vi "Sequence-Start tracking.vi"   [LabVIEW 2020]
uses:
  Global Variables/gl_UI Ctrl Refs.vi
types:
  T1 = enum8{"Enabled", "Disabled", "Disabled and Grayed Out"}
  T2 = typedef "UI ctrl refs cluster.ctl" = cluster{"Top level VI path":path, "Top level VI ref":refnum<vi>, "User menu ref":refnum<k9>, "Sub Panel control":refnum<vi>, "Imaging Param Tab":refnum<vi>, "Occurrence-Start drivers":refnum<k4>, "Occurrence-Speed logging initialised":refnum<k4>, "Occurrence-XYZ stage initialised":refnum<k4>, "Exit button":refnum<vi>, "Status ind":refnum<vi>, "Set as origin":refnum<vi>, "Speed Logging":refnum<vi>, "Time Lapse":refnum<vi>, "Live Imaging":refnum<vi>, "AOL Z Stack":refnum<vi>, "Motor Z Stack":refnum<vi>, "Funct Acq button":refnum<vi>, "Hard Shutter":refnum<vi>, "Virtual Shutter":refnum<vi>, "Laser Power":refnum<vi>, "AOL Mode":refnum<vi>, "Frame Size":refnum<vi>, "Field of View":refnum<vi>, "Dwell Time":refnum<vi>, "Zoom":refnum<vi>, "AOL Z":refnum<vi>, "Objective":refnum<vi>, "Axis":refnum<vi>, "Paths & Names":refnum<vi>, "Experiment folder path (ind.)":refnum<vi>, "Last State (Ind.)":refnum<vi>, "Averages":refnum<vi>, "Angle (degrees)":refnum<vi>, "X centre":refnum<vi>, "Y centre":refnum<vi>, "Plane Mode":refnum<vi>, "# Planes":refnum<vi>, "Z Start":refnum<vi>, "Z Stop":refnum<vi>, "Z Step":refnum<vi>, "PMT 1":refnum<vi>, "PMT 2":refnum<vi>, "Stage XYZ Position":refnum<vi>, "Pockels@Z Start":refnum<vi>, "Pockels@Z Stop":refnum<vi>, "Obtain Z Start":refnum<vi>, "Obtain Z Stop":refnum<vi>, "Live stim.trig.period":refnum<vi>, "Live stim.trig.enable":refnum<vi>, "Movement Correction":refnum<vi>, "Load Reference Image":refnum<vi>, "XY Stage Move":refnum<vi>, "MovCor Cluster":refnum<vi>, "RefDAQParam":refnum<vi>, "Funct. Acq. Pockels Modulation":refnum<vi>, "Ref Laser Power":refnum<vi>, "Enable Video Recording":refnum<vi>, "Video Record-Live Imaging":refnum<vi>, "Video Record-Funct acq":refnum<vi>, "Reference Source":refnum<vi>, "AOL Z-stack Chirps Ready (ind)":refnum<vi>, "Target time between mov.cor. ref triggers (ms)":refnum<vi>, "Funct. Acq. Ref frame save":refnum<vi>, "Tracking button":refnum<vi>, "Show ref plots window":refnum<vi>, "Center freq ind (nm)":refnum<vi>, "Pickup mode (ind)":refnum<vi>, "Logging queue (ind)":refnum<vi>, "Back aperture power (ind.)":refnum<vi>, "Power after objective (ind.)":refnum<vi>, "Switch user":refnum<vi>, "Ls1 Conn. Status":refnum<vi>, "Ls1Tuning Status":refnum<vi>, "Ls1 Faults":refnum<vi>, "Ls1 Connection":refnum<vi>, "Ls1 Mode":refnum<vi>, "Ls1 POWER [mW]":refnum<vi>, "Ls1Shutter":refnum<vi>, "Ls1 Wavelength":refnum<vi>, "Ls1 Note":refnum<vi>, "Ls1 Confirm Wav":refnum<vi>, "Ls1 PreChrp Prism1":refnum<vi>, "Ls1 PreChrp Prism2":refnum<vi>, "Ls1 wav top Ind":refnum<vi>, "Ls1 power top Ind":refnum<vi>, "Ls1 Pump peak Hold":refnum<vi>, "Ls1 Status Ind":refnum<vi>, "Ls1 wav cancel":refnum<vi>, "Experiment Type":refnum<vi>, "Biology Information":refnum<vi>, "Camera recording status":refnum<vi>}
  T3 = typedef "test_fpga_control.ctl" = cluster{"x_offset_host":fxp<+/-,16,8>, "y_offset_host":fxp<+/-,16,8>, "use host offset":bool, "Set_Ref_Centroid":bool, "OldChirpCode":bool, "use array of offsets":bool, "x_offset_host array":fxp<+/-,16,8>[], "y_offset_host array ":fxp<+/-,16,8>[], "use host offset Z":bool, "swap Z":bool, "z_offset_host ":fxp<+/-,16,8>}
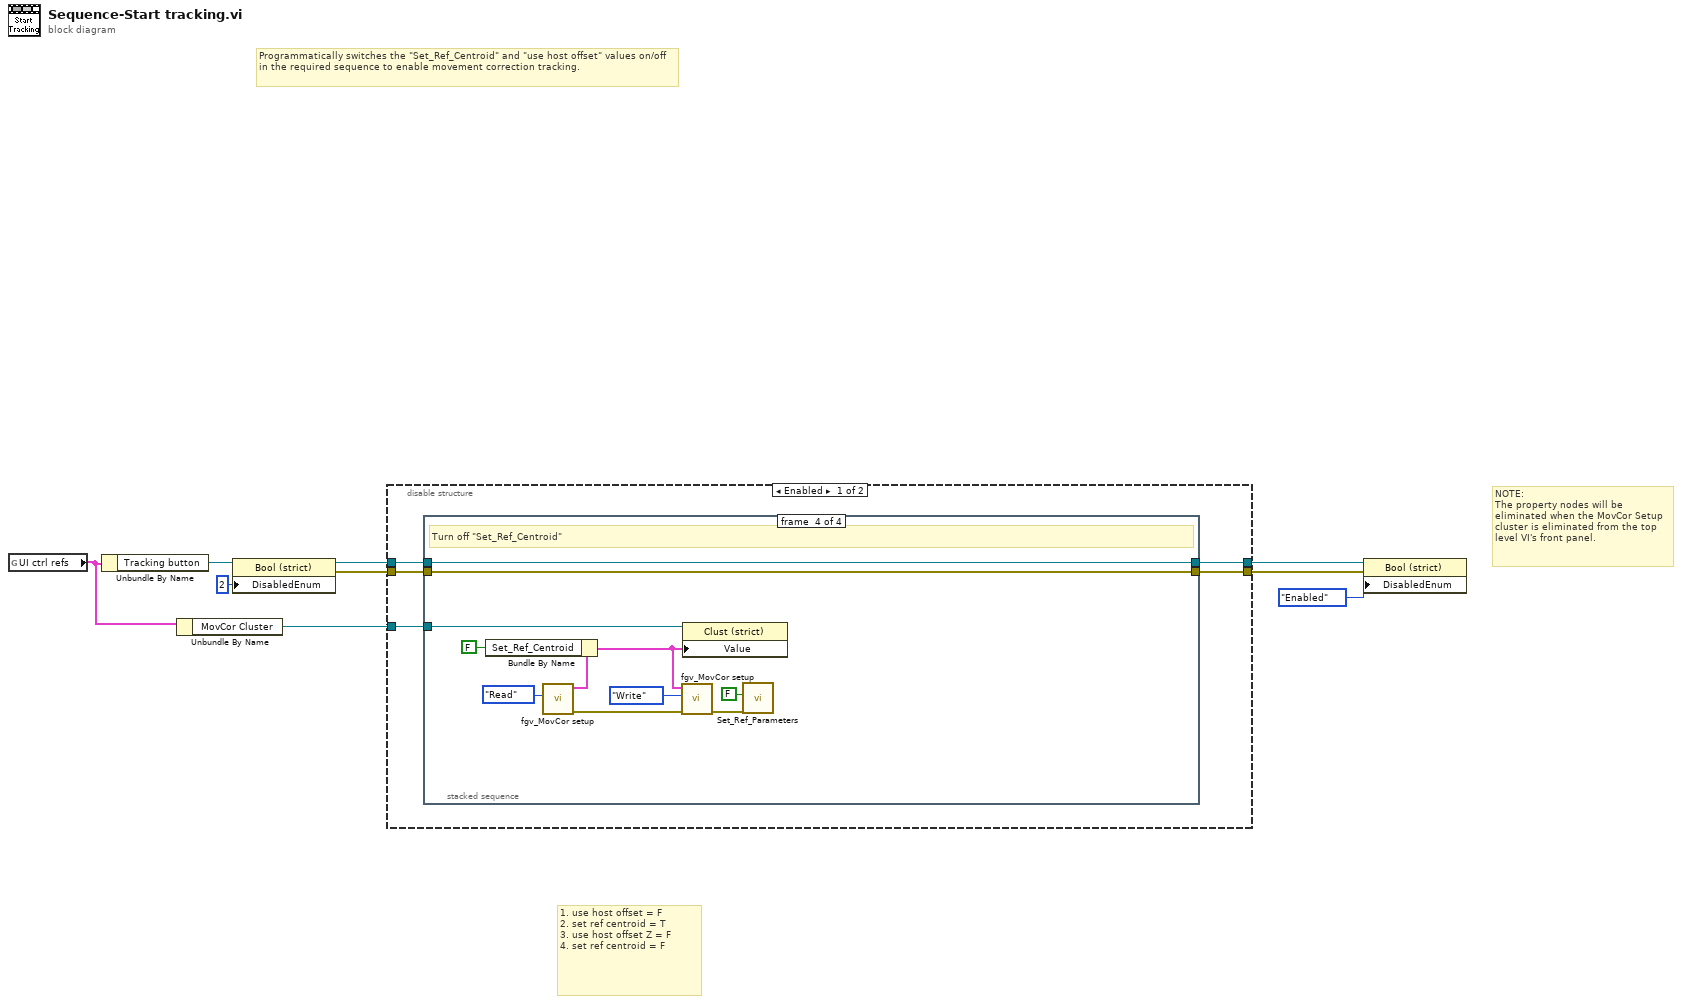
[diagram p0: block diagram]
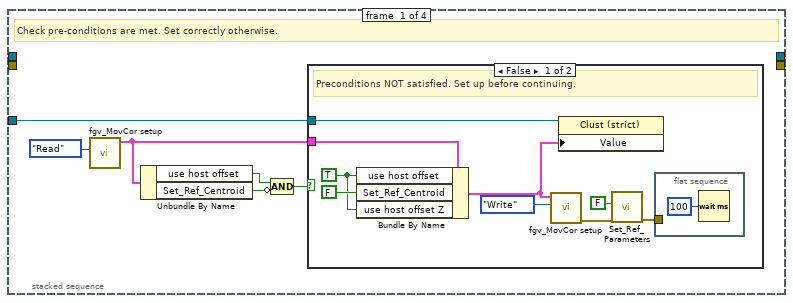
[diagram p2: hidden frame]
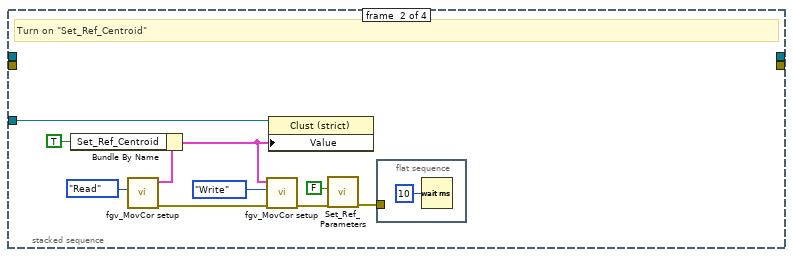
[diagram p4: hidden frame]
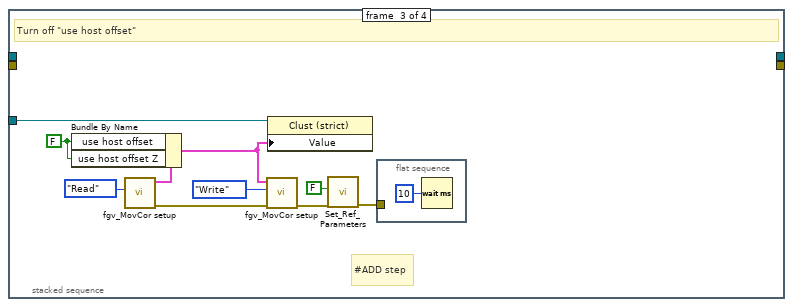
[diagram p5: hidden frame]
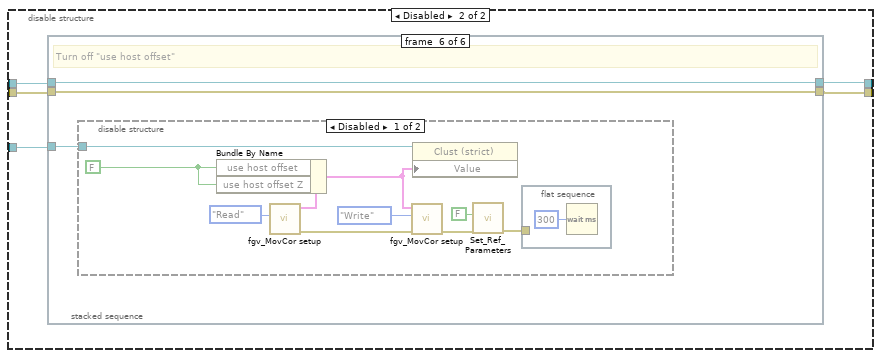
[diagram p6: hidden frame]
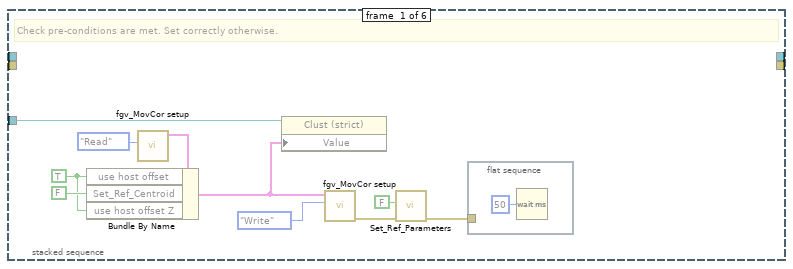
[diagram p7: hidden frame]
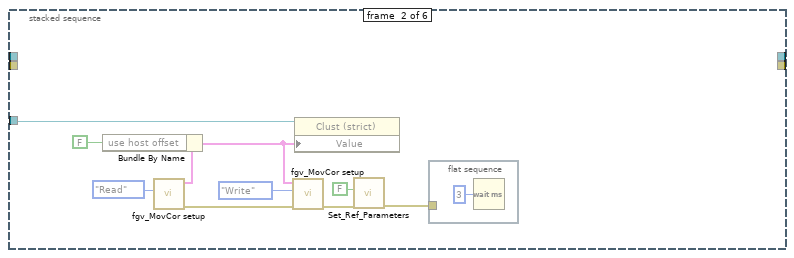
[diagram p8: hidden frame]
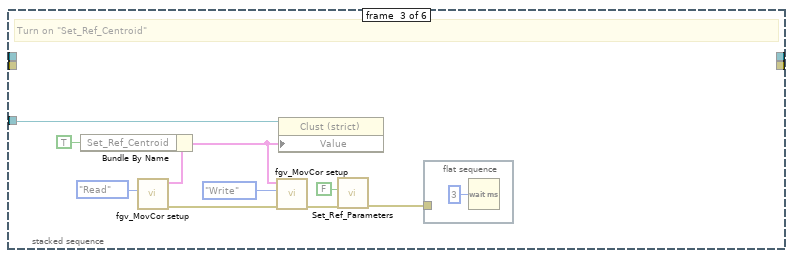
[diagram p9: hidden frame]
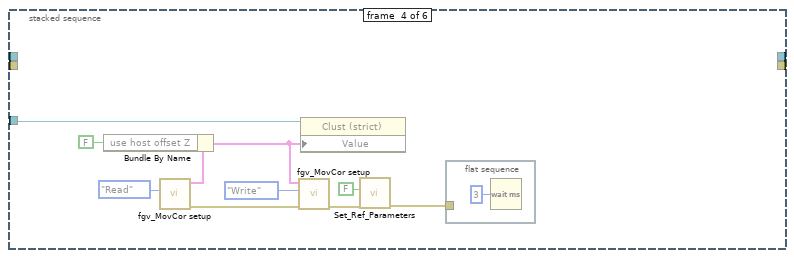
[diagram p10: hidden frame]
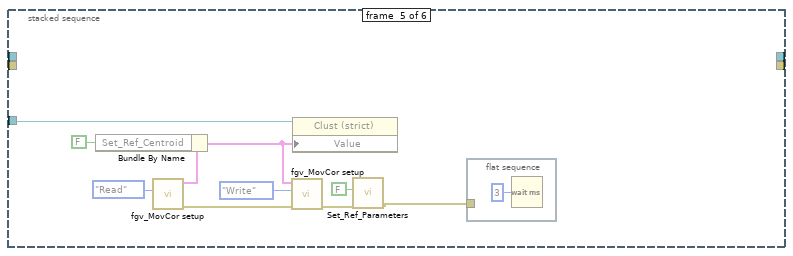
[diagram p11: hidden frame]
diagram:
  # "1. use host offset = F\n2. set ref centroid = T\n3. use host offset Z = F\n4. set ref centroid = F"
  # "NOTE:\nThe property nodes will be eliminated when the MovCor Setup cluster is eliminated from the top level VI's front panel."
  # "Programmatically switches the \"Set_Ref_Centroid\" and \"use host offset\" values on/off in the required sequence to enable movement correction tracking."
  n1 = global read "gl_UI Ctrl Refs.vi" "UI ctrl refs"() -> (w2:T2)
  n2 = Unbundle By Name(w2) -> ("Tracking button"=w3:refnum<vi>)
  n3 = Unbundle By Name(w2) -> ("MovCor Cluster"=w9:refnum<vi>)
  n4 = property on="Property Node" class="Bool (strict)"(reference=w3, "DisabledEnum"=2) -> (reference out=w6:refnum<vi>, error out=w7:errorcluster)  [unwired: 1 in]
  n5 = disable-structure shown="Enabled" {
    disable-tunnel: w9 -> [w14 w66]
    disable-tunnel: w7 -> [w13 w67]
    disable-tunnel: w6 -> [w12 w68]
    disable-tunnel: [w11 w65] -> w5
    disable-tunnel: [w10 w64] -> w4
    frame Enabled {
      n6 = stacked-sequence {
        tunnel: w14 -> [w15 w33 w45 w57]
        tunnel: w13 -> [_ _ _ w53]
        tunnel: [_ _ _ w54] -> w11
        tunnel: w12 -> [_ _ _ w54]
        tunnel: [_ _ _ w53] -> w10
        frame #0 {
          # "Check pre-conditions are met. Set correctly otherwise."
          n7 = call "fgv_MovCor setup.vi"("Status"=enum16{"Initialize", "Write", "Read"}."Read") -> ("MovCor Cluster"=w16:T3)  [unwired: 9 in, 1 out]
          n8 = Unbundle By Name(w16) -> ("use host offset"=w20:bool, "Set_Ref_Centroid"=w19:bool)
          n9 = Compound Arithmetic op=AND(w20, invert w19) -> (w18:bool)
          n10 = case shown="False" w18 {
            tunnel: w16 -> [w28 _]
            tunnel: w15 -> [w22 _]
            frame False {
              w21 = TRUE ("use host offset")
              # "Preconditions NOT satisfied. Set up before continuing."
              n11 = Bundle By Name(cluster=w28, "use host offset"=w21, "Set_Ref_Centroid"=FALSE, "use host offset Z"=w21) -> (w23:T3)
              n12 = call "fgv_MovCor setup.vi"("Status"=enum16{"Initialize", "Write", "Read"}."Write", "MovCor Cluster"=w23) -> ("error out"=w25:errorcluster)  [unwired: 8 in, 1 out]
              n13 = property class="Clust (strict)"(reference=w22, "Value"=w23) -> ()  [unwired: 1 in, 2 out]
              n14 = call "Set_Ref_Parameters.vi"("error in"=w25, "use_increment_halfrate"=FALSE) -> ("error out"=w24:errorcluster)  [unwired: 7 in, 2 out]
              n15 = flat-sequence {
                tunnel: w24 -> [_]
                frame #0 {
                  n16 = Wait (ms)(milliseconds to wait=u32 100 ("millisecond multiple")) -> ()  [unwired: 1 out]
                }
              }
            }
            frame True {
              # "Preconditions satisfied to allow continuing"
            }
          }
        }
        frame #1 {
          # "Turn on \"Set_Ref_Centroid\""
          n17 = call "fgv_MovCor setup.vi"("Status"=enum16{"Initialize", "Write", "Read"}."Read") -> ("error out"=w31:errorcluster, "MovCor Cluster"=w34:T3)  [unwired: 9 in]
          n18 = Bundle By Name(cluster=w34, "Set_Ref_Centroid"=TRUE) -> (w32:T3)
          n19 = call "fgv_MovCor setup.vi"("error in (no error)"=w31, "Status"=enum16{"Initialize", "Write", "Read"}."Write", "MovCor Cluster"=w32) -> ("error out"=w37:errorcluster)  [unwired: 7 in, 1 out]
          n20 = property class="Clust (strict)"(reference=w33, "Value"=w32) -> ()  [unwired: 1 in, 2 out]
          n21 = call "Set_Ref_Parameters.vi"("error in"=w37, "use_increment_halfrate"=FALSE) -> ("error out"=w40:errorcluster)  [unwired: 7 in, 2 out]
          n22 = flat-sequence {
            tunnel: w40 -> [_]
            frame #0 {
              n23 = Wait (ms)(milliseconds to wait=u32 10 ("millisecond multiple")) -> ()  [unwired: 1 out]
            }
          }
        }
        frame #2 {
          w42 = FALSE ("Set_Ref_Centroid")
          # "#ADD step"
          # "Turn off \"use host offset\""
          n24 = call "fgv_MovCor setup.vi"("Status"=enum16{"Initialize", "Write", "Read"}."Read") -> ("error out"=w43:errorcluster, "MovCor Cluster"=w46:T3)  [unwired: 9 in]
          n25 = Bundle By Name(cluster=w46, "use host offset"=w42, "use host offset Z"=w42) -> (w44:T3)
          n26 = call "fgv_MovCor setup.vi"("error in (no error)"=w43, "Status"=enum16{"Initialize", "Write", "Read"}."Write", "MovCor Cluster"=w44) -> ("error out"=w48:errorcluster)  [unwired: 7 in, 1 out]
          n27 = property class="Clust (strict)"(reference=w45, "Value"=w44) -> ()  [unwired: 1 in, 2 out]
          n28 = call "Set_Ref_Parameters.vi"("error in"=w48, "use_increment_halfrate"=FALSE) -> ("error out"=w51:errorcluster)  [unwired: 7 in, 2 out]
          n29 = flat-sequence {
            tunnel: w51 -> [_]
            frame #0 {
              n30 = Wait (ms)(milliseconds to wait=u32 10 ("millisecond multiple")) -> ()  [unwired: 1 out]
            }
          }
        }
        frame #3 {
          # "Turn off \"Set_Ref_Centroid\""
          n31 = call "fgv_MovCor setup.vi"("Status"=enum16{"Initialize", "Write", "Read"}."Read") -> ("error out"=w55:errorcluster, "MovCor Cluster"=w58:T3)  [unwired: 9 in]
          n32 = Bundle By Name(cluster=w58, "Set_Ref_Centroid"=FALSE) -> (w56:T3)
          n33 = call "fgv_MovCor setup.vi"("error in (no error)"=w55, "Status"=enum16{"Initialize", "Write", "Read"}."Write", "MovCor Cluster"=w56) -> ("error out"=w61:errorcluster)  [unwired: 7 in, 1 out]
          n34 = property class="Clust (strict)"(reference=w57, "Value"=w56) -> ()  [unwired: 1 in, 2 out]
          n35 = call "Set_Ref_Parameters.vi"("error in"=w61, "use_increment_halfrate"=FALSE) -> ()  [unwired: 7 in, 3 out]
        }
      }
    }
    frame Disabled {
      n36 = stacked-sequence {
        tunnel: w66 -> [w76 w80 w93 w102 w114 w126]
        tunnel: w67 -> [_ _ _ _ _ w124]
        tunnel: [_ _ _ _ _ w125] -> w65
        tunnel: w68 -> [_ _ _ _ _ w125]
        tunnel: [_ _ _ _ _ w124] -> w64
        frame #0 {
          w73 = TRUE ("use host offset")
          # "Check pre-conditions are met. Set correctly otherwise."
          n37 = call "fgv_MovCor setup.vi"("Status"=enum16{"Initialize", "Write", "Read"}."Read") -> ("MovCor Cluster"=w77:T3)  [unwired: 9 in, 1 out]
          n38 = Bundle By Name(cluster=w77, "use host offset"=w73, "Set_Ref_Centroid"=FALSE, "use host offset Z"=w73) -> (w74:T3)
          n39 = property class="Clust (strict)"(reference=w76, "Value"=w74) -> ()  [unwired: 1 in, 2 out]
          n40 = call "fgv_MovCor setup.vi"("Status"=enum16{"Initialize", "Write", "Read"}."Write", "MovCor Cluster"=w74) -> ("error out"=w72:errorcluster)  [unwired: 8 in, 1 out]
          n41 = call "Set_Ref_Parameters.vi"("error in"=w72, "use_increment_halfrate"=FALSE) -> ("error out"=w69:errorcluster)  [unwired: 7 in, 2 out]
          n42 = flat-sequence {
            tunnel: w69 -> [_]
            frame #0 {
              n43 = Wait (ms)(milliseconds to wait=u32 50 ("millisecond multiple")) -> ()  [unwired: 1 out]
            }
          }
        }
        frame #1 {
          n44 = call "fgv_MovCor setup.vi"("Status"=enum16{"Initialize", "Write", "Read"}."Read") -> ("error out"=w81:errorcluster, "MovCor Cluster"=w83:T3)  [unwired: 9 in]
          n45 = Bundle By Name(cluster=w83, "use host offset"=FALSE ("Set_Ref_Centroid")) -> (w82:T3)
          n46 = call "fgv_MovCor setup.vi"("error in (no error)"=w81, "Status"=enum16{"Initialize", "Write", "Read"}."Write", "MovCor Cluster"=w82) -> ("error out"=w86:errorcluster)  [unwired: 7 in, 1 out]
          n47 = property class="Clust (strict)"(reference=w80, "Value"=w82) -> ()  [unwired: 1 in, 2 out]
          n48 = call "Set_Ref_Parameters.vi"("error in"=w86, "use_increment_halfrate"=FALSE) -> ("error out"=w89:errorcluster)  [unwired: 7 in, 2 out]
          n49 = flat-sequence {
            tunnel: w89 -> [_]
            frame #0 {
              n50 = Wait (ms)(milliseconds to wait=u32 3 ("millisecond multiple")) -> ()  [unwired: 1 out]
            }
          }
        }
        frame #2 {
          # "Turn on \"Set_Ref_Centroid\""
          n51 = call "fgv_MovCor setup.vi"("Status"=enum16{"Initialize", "Write", "Read"}."Read") -> ("error out"=w91:errorcluster, "MovCor Cluster"=w94:T3)  [unwired: 9 in]
          n52 = Bundle By Name(cluster=w94, "Set_Ref_Centroid"=TRUE) -> (w92:T3)
          n53 = call "fgv_MovCor setup.vi"("error in (no error)"=w91, "Status"=enum16{"Initialize", "Write", "Read"}."Write", "MovCor Cluster"=w92) -> ("error out"=w97:errorcluster)  [unwired: 7 in, 1 out]
          n54 = property class="Clust (strict)"(reference=w93, "Value"=w92) -> ()  [unwired: 1 in, 2 out]
          n55 = call "Set_Ref_Parameters.vi"("error in"=w97, "use_increment_halfrate"=FALSE) -> ("error out"=w100:errorcluster)  [unwired: 7 in, 2 out]
          n56 = flat-sequence {
            tunnel: w100 -> [_]
            frame #0 {
              n57 = Wait (ms)(milliseconds to wait=u32 3 ("millisecond multiple")) -> ()  [unwired: 1 out]
            }
          }
        }
        frame #3 {
          n58 = call "fgv_MovCor setup.vi"("Status"=enum16{"Initialize", "Write", "Read"}."Read") -> ("error out"=w103:errorcluster, "MovCor Cluster"=w105:T3)  [unwired: 9 in]
          n59 = Bundle By Name(cluster=w105, "use host offset Z"=FALSE ("Set_Ref_Centroid")) -> (w104:T3)
          n60 = call "fgv_MovCor setup.vi"("error in (no error)"=w103, "Status"=enum16{"Initialize", "Write", "Read"}."Write", "MovCor Cluster"=w104) -> ("error out"=w108:errorcluster)  [unwired: 7 in, 1 out]
          n61 = property class="Clust (strict)"(reference=w102, "Value"=w104) -> ()  [unwired: 1 in, 2 out]
          n62 = call "Set_Ref_Parameters.vi"("error in"=w108, "use_increment_halfrate"=FALSE) -> ("error out"=w111:errorcluster)  [unwired: 7 in, 2 out]
          n63 = flat-sequence {
            tunnel: w111 -> [_]
            frame #0 {
              n64 = Wait (ms)(milliseconds to wait=u32 3 ("millisecond multiple")) -> ()  [unwired: 1 out]
            }
          }
        }
        frame #4 {
          n65 = call "fgv_MovCor setup.vi"("Status"=enum16{"Initialize", "Write", "Read"}."Read") -> ("error out"=w115:errorcluster, "MovCor Cluster"=w117:T3)  [unwired: 9 in]
          n66 = Bundle By Name(cluster=w117, "Set_Ref_Centroid"=FALSE) -> (w116:T3)
          n67 = call "fgv_MovCor setup.vi"("error in (no error)"=w115, "Status"=enum16{"Initialize", "Write", "Read"}."Write", "MovCor Cluster"=w116) -> ("error out"=w120:errorcluster)  [unwired: 7 in, 1 out]
          n68 = property class="Clust (strict)"(reference=w114, "Value"=w116) -> ()  [unwired: 1 in, 2 out]
          n69 = call "Set_Ref_Parameters.vi"("error in"=w120, "use_increment_halfrate"=FALSE) -> ("error out"=w113:errorcluster)  [unwired: 7 in, 2 out]
          n70 = flat-sequence {
            tunnel: w113 -> [_]
            frame #0 {
              n71 = Wait (ms)(milliseconds to wait=u32 3 ("millisecond multiple")) -> ()  [unwired: 1 out]
            }
          }
        }
        frame #5 {
          # "Turn off \"use host offset\""
          n72 = disable-structure shown="Disabled" {
            disable-tunnel: w126 -> [w130 _]
            frame Disabled {
              w127 = FALSE ("Set_Ref_Centroid")
              n73 = call "fgv_MovCor setup.vi"("Status"=enum16{"Initialize", "Write", "Read"}."Read") -> ("error out"=w128:errorcluster, "MovCor Cluster"=w131:T3)  [unwired: 9 in]
              n74 = Bundle By Name(cluster=w131, "use host offset"=w127, "use host offset Z"=w127) -> (w129:T3)
              n75 = call "fgv_MovCor setup.vi"("error in (no error)"=w128, "Status"=enum16{"Initialize", "Write", "Read"}."Write", "MovCor Cluster"=w129) -> ("error out"=w133:errorcluster)  [unwired: 7 in, 1 out]
              n76 = property class="Clust (strict)"(reference=w130, "Value"=w129) -> ()  [unwired: 1 in, 2 out]
              n77 = call "Set_Ref_Parameters.vi"("error in"=w133, "use_increment_halfrate"=FALSE) -> ("error out"=w136:errorcluster)  [unwired: 7 in, 2 out]
              n78 = flat-sequence {
                tunnel: w136 -> [_]
                frame #0 {
                  n79 = Wait (ms)(milliseconds to wait=u32 300 ("millisecond multiple")) -> ()  [unwired: 1 out]
                }
              }
            }
            frame Enabled {
            }
          }
        }
      }
    }
  }
  n80 = property on="Property Node" class="Bool (strict)"(reference=w5, error in=w4, "DisabledEnum"=T1."Enabled" ("Disabled")) -> ()  [unwired: 2 out]
